vi "Initialize.vi"(8 "error in (no error)":errorcluster, 10 "logger name":string, 11 "handler in":refnum<class "Formatting Handler.lvclass">) -> (0 "error out":errorcluster, 2 "handler name":string, 3 "handler out":refnum<class "Formatting Handler.lvclass">)   [LabVIEW 2018, in "GLog.lvlib" / "Formatting Handler.lvclass"]
uses:
  Formatting Handler.lvclass
  Formatting Handler.lvclass/Formatting Handler.ctl
panel:
  # "Connector Pane"
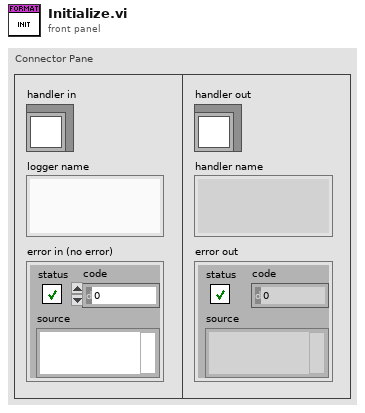
[diagram p1: front panel]
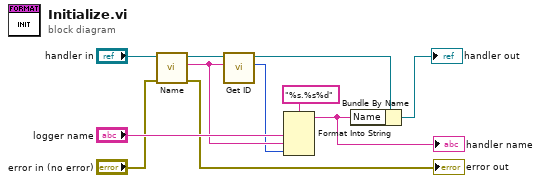
[diagram p0: block diagram]
diagram:
  n1 = call-dynamic "Name.vi"("error in (no error)"="error in (no error)", "Formatting Handler in"="handler in") -> ("error out"=→"error out":errorcluster, "class name"=w4:string, "Formatting Handler out"=w3:refnum<class "Formatting Handler.lvclass">)  [unwired: 7 in]
  n2 = call "Get ID.vi"("name"=w4, "Formatting Handler in"=w3) -> ("ID"=w1:i32, "Formatting Handler out"=w2:refnum<class "Formatting Handler.lvclass">)  [unwired: 7 in, 1 out]
  n3 = Format Into String(format string="%s.%s%d", "logger name", w4, w1) -> (resulting string=w8:string)  [unwired: 2 in, 1 out]
  "handler name" <- w8
  n4 = Bundle By Name(cluster=w2, "Name"=w8) -> (→"handler out":refnum<class "Formatting Handler.lvclass">)
